vi "Get Control References And Add To DVR.vi"(6 "Controls[]":refnum<vi>[](array[refnum]), 8 "error in (no error)":errorcluster) -> (0 "error out":errorcluster)   [LabVIEW 2019, in "Language Selection.lvlib"]
doc: "This reentrant VI will get the references of all the controls contained in the VI´s front panel.\n- - -\nCopyright (c) 2026, Merecs Engineering GmbH"
uses:
  Language Selection.lvlib
  Global Language Selection.vi
panel:
  # "Connector Pane"
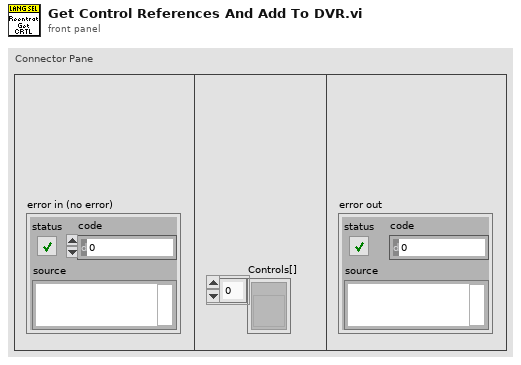
[diagram p1: front panel]
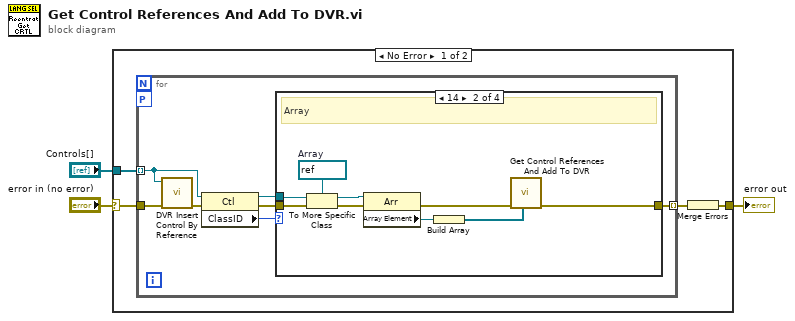
[diagram p0: block diagram]
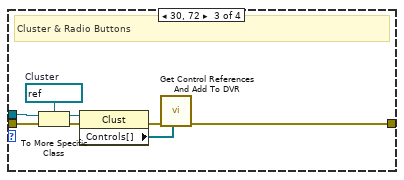
[diagram p3: hidden frame]
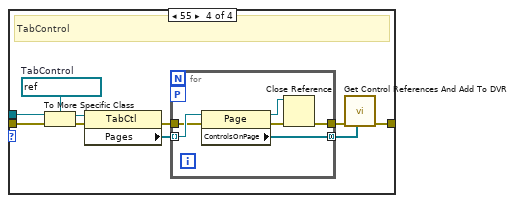
[diagram p4: hidden frame]
diagram:
  n1 = case shown="No Error" "error in (no error)" {
    selector: "error in (no error)" -> [w5 w49]
    tunnel: [w4 w49] -> w1
    tunnel: "Controls[]" -> [w6 _]
    frame No Error {
      n2 = for {
        tunnel: [w8] -> w7 mode=indexing
        tunnel: w6 -> [w11] mode=indexing
        tunnel: w5 -> [w10]
        workers-P: _ -> [_]
        n3 = call "DVR Insert Control By Reference.vi"("error in (no error)"=w10, "Ctl Refnum"=w11) -> ("error out"=w9:errorcluster)  [unwired: 9 in]
        n4 = property class="Ctl"(reference=w11, error in=w9) -> (reference out=w12:refnum<vi>, error out=w14:errorcluster, "ClassID"=w13:u32)
        n5 = case shown="14" w13 {
          tunnel: w12 -> [_ w24 w32 w42]
          tunnel: w14 -> [w15 w23 w31 w41]
          tunnel: [w15 w22 w30 w40] -> w8
          frame 0, Default {
          }
          frame 14 {
            w19 = refnum<vi> refnum  # Array
            # "Array"
            n6 = To More Specific Class(target class=w19, reference=w24, error in=w23) -> (specific class reference=w16:refnum<vi>, error out=w20:errorcluster)
            n7 = property class="Arr"(reference=w16, error in=w20) -> (error out=w21:errorcluster, "Array Element"=w18:refnum<vi>)  [unwired: 1 out]
            n8 = Build Array(w18) -> (w17:refnum<vi>[])
            n9 = call "Get Control References And Add To DVR.vi"("Controls[]"=w17, "error in (no error)"=w21) -> ("error out"=w22:errorcluster)  [unwired: 9 in]
          }
          frame 30, 72 {
            w26 = refnum<vi> refnum  # Cluster
            # "Cluster & Radio Buttons"
            n10 = To More Specific Class(target class=w26, reference=w32, error in=w31) -> (specific class reference=w25:refnum<vi>, error out=w27:errorcluster)
            n11 = property class="Clust"(reference=w25, error in=w27) -> (error out=w28:errorcluster, "Controls[]"=w29:refnum<vi>[])  [unwired: 1 out]
            n12 = call "Get Control References And Add To DVR.vi"("Controls[]"=w29, "error in (no error)"=w28) -> ("error out"=w30:errorcluster)  [unwired: 9 in]
          }
          frame 55 {
            w37 = refnum<vi> refnum  # TabControl
            # "TabControl"
            n13 = To More Specific Class(target class=w37, reference=w42, error in=w41) -> (specific class reference=w33:refnum<vi>, error out=w38:errorcluster)
            n14 = property class="TabCtl"(reference=w33, error in=w38) -> (error out=w39:errorcluster, "Pages"=w35:refnum<vi>[])  [unwired: 1 out]
            n15 = for {
              tunnel: [w44] -> w36
              tunnel: w39 -> [w46]
              tunnel: w35 -> [w47] mode=indexing
              tunnel: [w48] -> w34 mode=concatenating
              workers-P: _ -> [_]
              n16 = property class="Page"(reference=w47, error in=w46) -> (reference out=w43:refnum<vi>, error out=w45:errorcluster, "ControlsOnPage"=w48:refnum<vi>[])
              n17 = Close Reference(reference=w43, error in (no error)=w45) -> (error out=w44:errorcluster)
            }
            n18 = call "Get Control References And Add To DVR.vi"("Controls[]"=w34, "error in (no error)"=w36) -> ("error out"=w40:errorcluster)  [unwired: 9 in]
          }
        }
      }
      n19 = Merge Errors(w7) -> (w4:errorcluster)
    }
    frame Error {
    }
  }
  "error out" <- w1
